vi "Generate Stream Event.vi"(6 "Session ID":i32, 7 "Direction":T1, 8 "error in (no error)":errorcluster, 10 "Bytes":u8[](array[numeric]) format="%02x", 11 "DebuggingTerminal in":refnum<class "DebuggingTerminal.lvclass">) -> (0 "error out":errorcluster, 3 "DebuggingTerminal out":refnum<class "DebuggingTerminal.lvclass">)   [LabVIEW 2013, in "MQTT Base.lvlib" / "DebuggingTerminal.lvclass"]
uses:
  DebuggingTerminal.lvclass
  Stream Direction -- enum.ctl
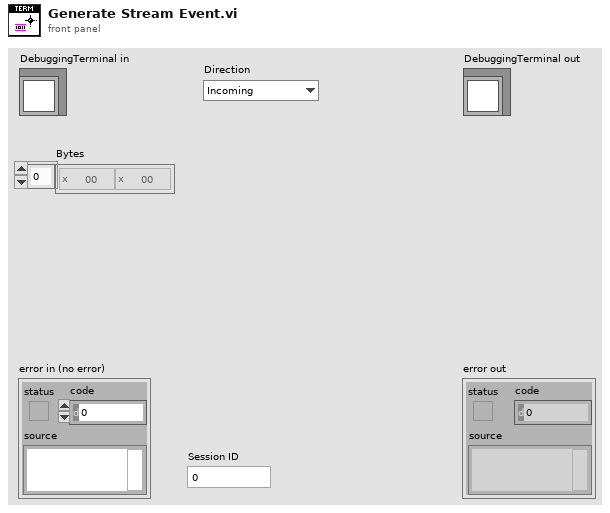
[diagram p1: front panel]
types:
  T1 = typedef "MQTT Base.lvlib/DebuggingTerminal.lvclass/Stream Direction -- enum.ctl" = enum16{"Incoming", "Outgoing"}
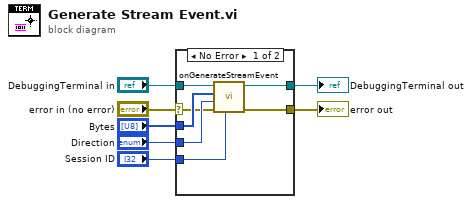
[diagram p0: block diagram]
diagram:
  n1 = case shown="No Error" "error in (no error)" {
    selector: "error in (no error)" -> [w10 w16]
    tunnel: [w9 w16] -> w6
    tunnel: [w11 w15] -> w4
    tunnel: "DebuggingTerminal in" -> [w12 w15]
    tunnel: "Bytes" -> [w14 _]
    tunnel: "Direction" -> [w13 _]
    tunnel: "Session ID" -> [w8 _]
    frame No Error {
      n2 = call-dynamic "onGenerateStreamEvent.vi"("Session ID"=w8, "error in (no error)"=w10, "Direction"=w13, "Bytes"=w14, "DebuggingTerminal in"=w12) -> ("error out"=w9:errorcluster, "DebuggingTerminal out"=w11:refnum<class "DebuggingTerminal.lvclass">)  [unwired: 5 in]
    }
    frame Error {
    }
  }
  "error out" <- w6
  "DebuggingTerminal out" <- w4
